vi "toNextMonth.vi"(7 "Values":i32[](array[numeric]), 11 "Cron in":T1) -> (3 "Cron out":T1)   [LabVIEW 2013, in "openCron.lvlib" / "Cron.lvclass"]
uses:
  Cron.lvclass
  CronTime -- cluster.ctl
  TimeStamp to Cron Time.vi
  Cron Time to TimeStamp.vi
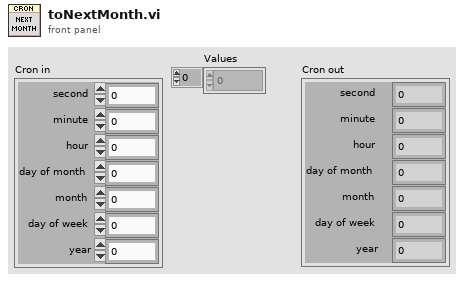
[diagram p1: front panel]
types:
  T1 = typedef "openCron.lvlib/Cron.lvclass/CronTime -- cluster.ctl" = cluster{"second":i32, "minute":i32, "hour":i32, "day of month":i32, "month":i32, "day of week":i32, "year":i32}
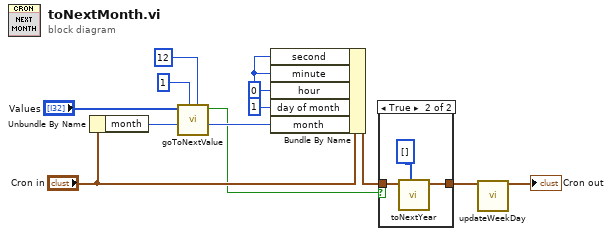
[diagram p0: block diagram]
diagram:
  w11 = 0 ("hour")
  n1 = Unbundle By Name("Cron in") -> ("month"=w5:i32)
  n2 = call "goToNextValue.vi"("maxValue"=12 ("upper limit"), "min Value"=1 ("lower limit"), "value in"=w5, "Values Pool"="Values") -> ("next value"=w2:i32, "RolledOver"=w1:bool)  [unwired: 6 in]
  n3 = Bundle By Name(cluster="Cron in", "second"=w11, "minute"=w11, "hour"=w11, "day of month"=1 ("month"), "month"=w2) -> (w9:T1)
  n4 = case shown="True" w1 {
    tunnel: w9 -> [w13 w16]
    tunnel: [w13 w15] -> w7
    frame False {
    }
    frame True {
      n5 = call "toNextYear.vi"("Values"=i32[] [], "Cron in"=w16) -> ("Cron out"=w15:T1)  [unwired: 9 in]
    }
  }
  n6 = call "updateWeekDay.vi"("Cron in"=w7) -> ("Cron Time"=→"Cron out":T1)  [unwired: 10 in]
